vi "laser_constant_current_output_with_DAQ_analog_output_timed.vi"() -> ()   [LabVIEW 2025, in "tSNIP.lvlib"]
uses:
  tSNIP.lvlib
panel:
  in  "error in (no error)":errorcluster
  out "error out":errorcluster
  in  "Timed?":bool
  in  "ON time":dbl format="%<%M:%S>t"
  out "Elapsed time":dbl format="%<%M:%S>t"
  in  "Power":cluster{"Value":dbl, "Units":dbl}={"Value"=0.0, "Units"=0.001} {"Units" items=["mW"=0.001, "W"=1.0]}
  in  "Current":cluster{"Value":dbl, "Units":dbl}={"Value"=0.0, "Units"=0.001} {"Units" items=["mA"=0.001, "A"=1.0]; "Value" min=0.0 max=2500.0 step=50.0}
  in  "DAQmx Device":tag
  in  "VISA resource name":refnum<visa-resource-name>
  in  "Laser Active":bool
  in  "STOP":bool
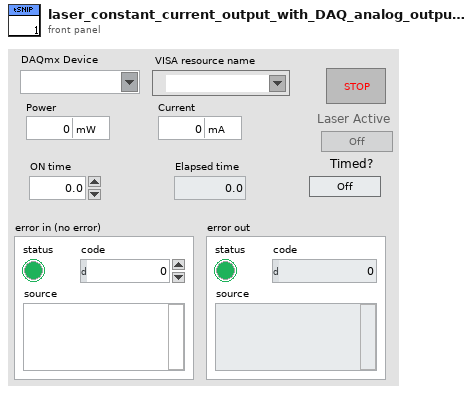
[diagram p1: front panel]
types:
  T1 = enum8{"Enabled", "Disabled", "Disabled and Grayed Out"}
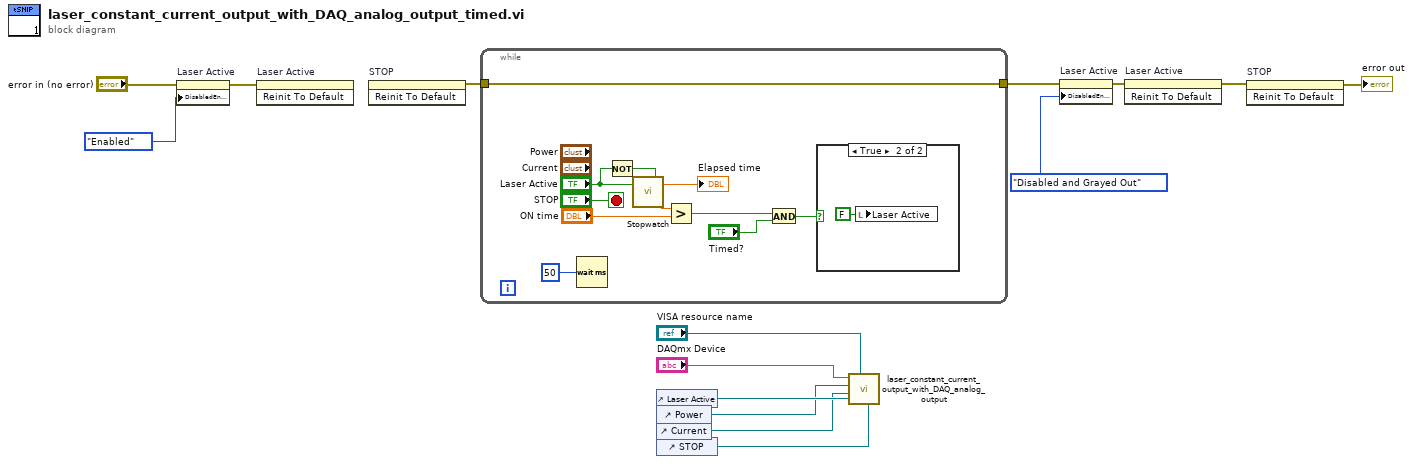
[diagram p0: block diagram]
diagram:
  n1 = property on="Laser Active" class="Bool (strict)"(error in="error in (no error)", "DisabledEnum"=T1."Enabled" ("Disabled")) -> (error out=w4:errorcluster)  [unwired: 1 in, 1 out]
  n2 = invoke on="Laser Active" class="Bool (strict)" method="Reinit To Default"(error in=w4) -> ()  [unwired: 2 in, 3 out]
  n3 = invoke on="STOP" class="Bool (strict)" method="Reinit To Default"() -> (error out=w9:errorcluster)  [unwired: 3 in, 2 out]
  n4 = while {
    tunnel: w9 -> [w16]
    tunnel: [w16] -> w7
    stop <- "STOP" stop-if-true
    n5 = Wait (ms)(milliseconds to wait=u32 50) -> ()  [unwired: 1 out]
    n6 = Not(x="Laser Active") -> (.not. x?=w25:bool)
    n7 = call "Stopwatch.vi"("Start"="Laser Active", "Reset"=w25) -> ("time"=w20:dbl)  [unwired: 17 in]
    "Elapsed time" <- w20
    n8 = Greater?(x=w20, y="ON time") -> (0:w23:bool)
    n9 = And(x=w23, y="Timed?") -> (x .and. y?=w18:bool)
    n10 = case shown="True" w18 {
      frame False {
      }
      frame True {
        n11 = local write "Laser Active"(FALSE) -> ()
      }
    }
  }
  n12 = control-ref of="Laser Active"() -> (w13:refnum<vi>)
  n13 = control-ref of="Power"() -> (w11:refnum<vi>)
  n14 = control-ref of="Current"() -> (w10:refnum<vi>)
  n15 = control-ref of="STOP"() -> (w12:refnum<vi>)
  n16 = call "laser_constant_current_output_with_DAQ_analog_output.vi"("Exit Refnum"=w12, "Activate Refnum"=w13, "VISA resource name"="VISA resource name", "Current Refnum"=w10, "Power Refnum"=w11, "DAQmx Device"="DAQmx Device") -> ()  [unwired: 5 in, 1 out]
  n17 = property on="Laser Active" class="Bool (strict)"(error in=w7, "DisabledEnum"=T1."Disabled and Grayed Out" ("Disabled")) -> (error out=w8:errorcluster)  [unwired: 1 in, 1 out]
  n18 = invoke on="Laser Active" class="Bool (strict)" method="Reinit To Default"(error in=w8) -> (error out=w2:errorcluster)  [unwired: 2 in, 2 out]
  n19 = invoke on="STOP" class="Bool (strict)" method="Reinit To Default"(error in=w2) -> (error out=→"error out":errorcluster)  [unwired: 2 in, 2 out]
